vi "10054_Control.vi"(5 "DO":bool caption="DO ON/OFF", 7 "error in":errorcluster, 8 "Operation":T1, 9 "Pin":T2=enum."Pilz-2", 10 "Resource In":refnum<visa-resource-name>) -> (0 "error out":errorcluster, 1 "Status":bool[](array[boolean]), 2 "Command Response":string, 3 "Resource out":refnum<visa-resource-name>)   [LabVIEW 2021]
uses:
  Support/10054_states.ctl
  Support/Relay_no.ctl
panel:
  # "UART TX"
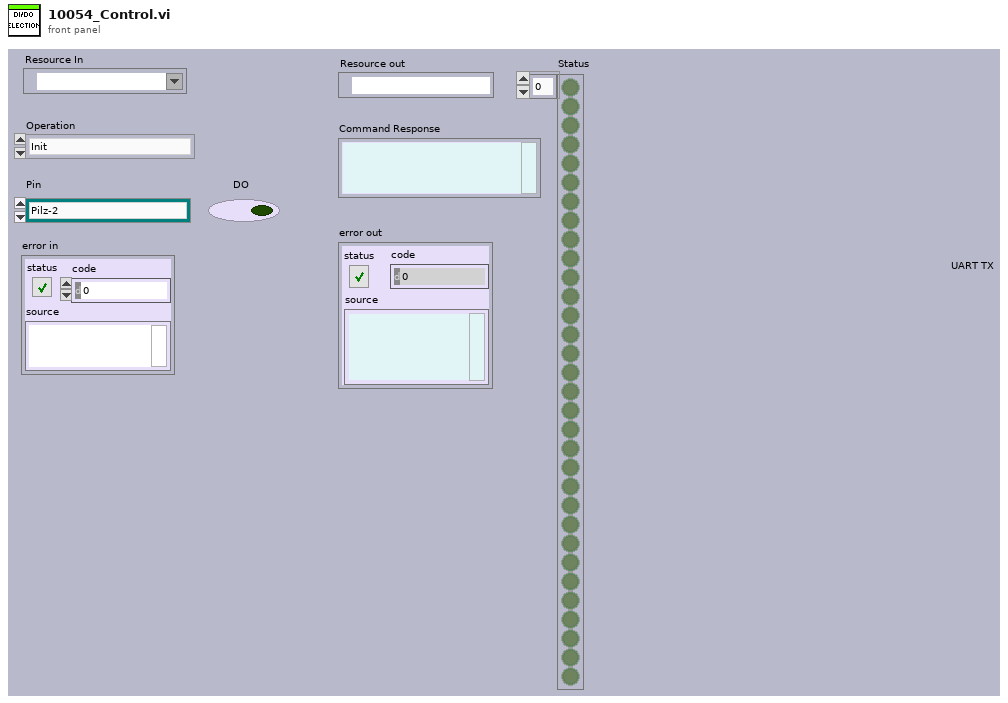
[diagram p1: front panel]
types:
  T1 = typedef "Relay_no.ctl" = enum16{"Init", "write&Read", "PCB Serial Write & Read", "PCB Write SSD & Password", "Read Wifi state", "Reset", "Close"}
  T2 = typedef "10054_states.ctl" = enum16{"Pilz-1", "Pilz-2", "AC CON - 2", "AC CON - 3", "AC CON - 4", "AC CON - 5", "Tower Lamp - Red", "Tower Lamp - Amber", "Tower Lamp - Green", "FAN 1 & 2", "FAN 3 & 4", "FAN 5 & 6", "Load - 1 10A", "Load - 2 10A", "Load - 3 5A", "Load - 4 5A", "Load - 5 2A", "TP49 - 12V", "TP20 - 5V", "TP148 - 3.3", "TP193 - GND", "J11.1 POS", "J11.2 NEG", "Noti LED POS", "Noti LED NEG", "Noti LED  5V", "D+M J14.1 - 3.3", "D+M J14.2 - GND", "NFC - 1", "NFC - 2"}
  T3 = cluster{"baud rate":u32, "data bits":u16, "parity":enum16{"None", "Odd", "Even", "Mark", "Space"}, "stop bits":u16, "flow control":u16}
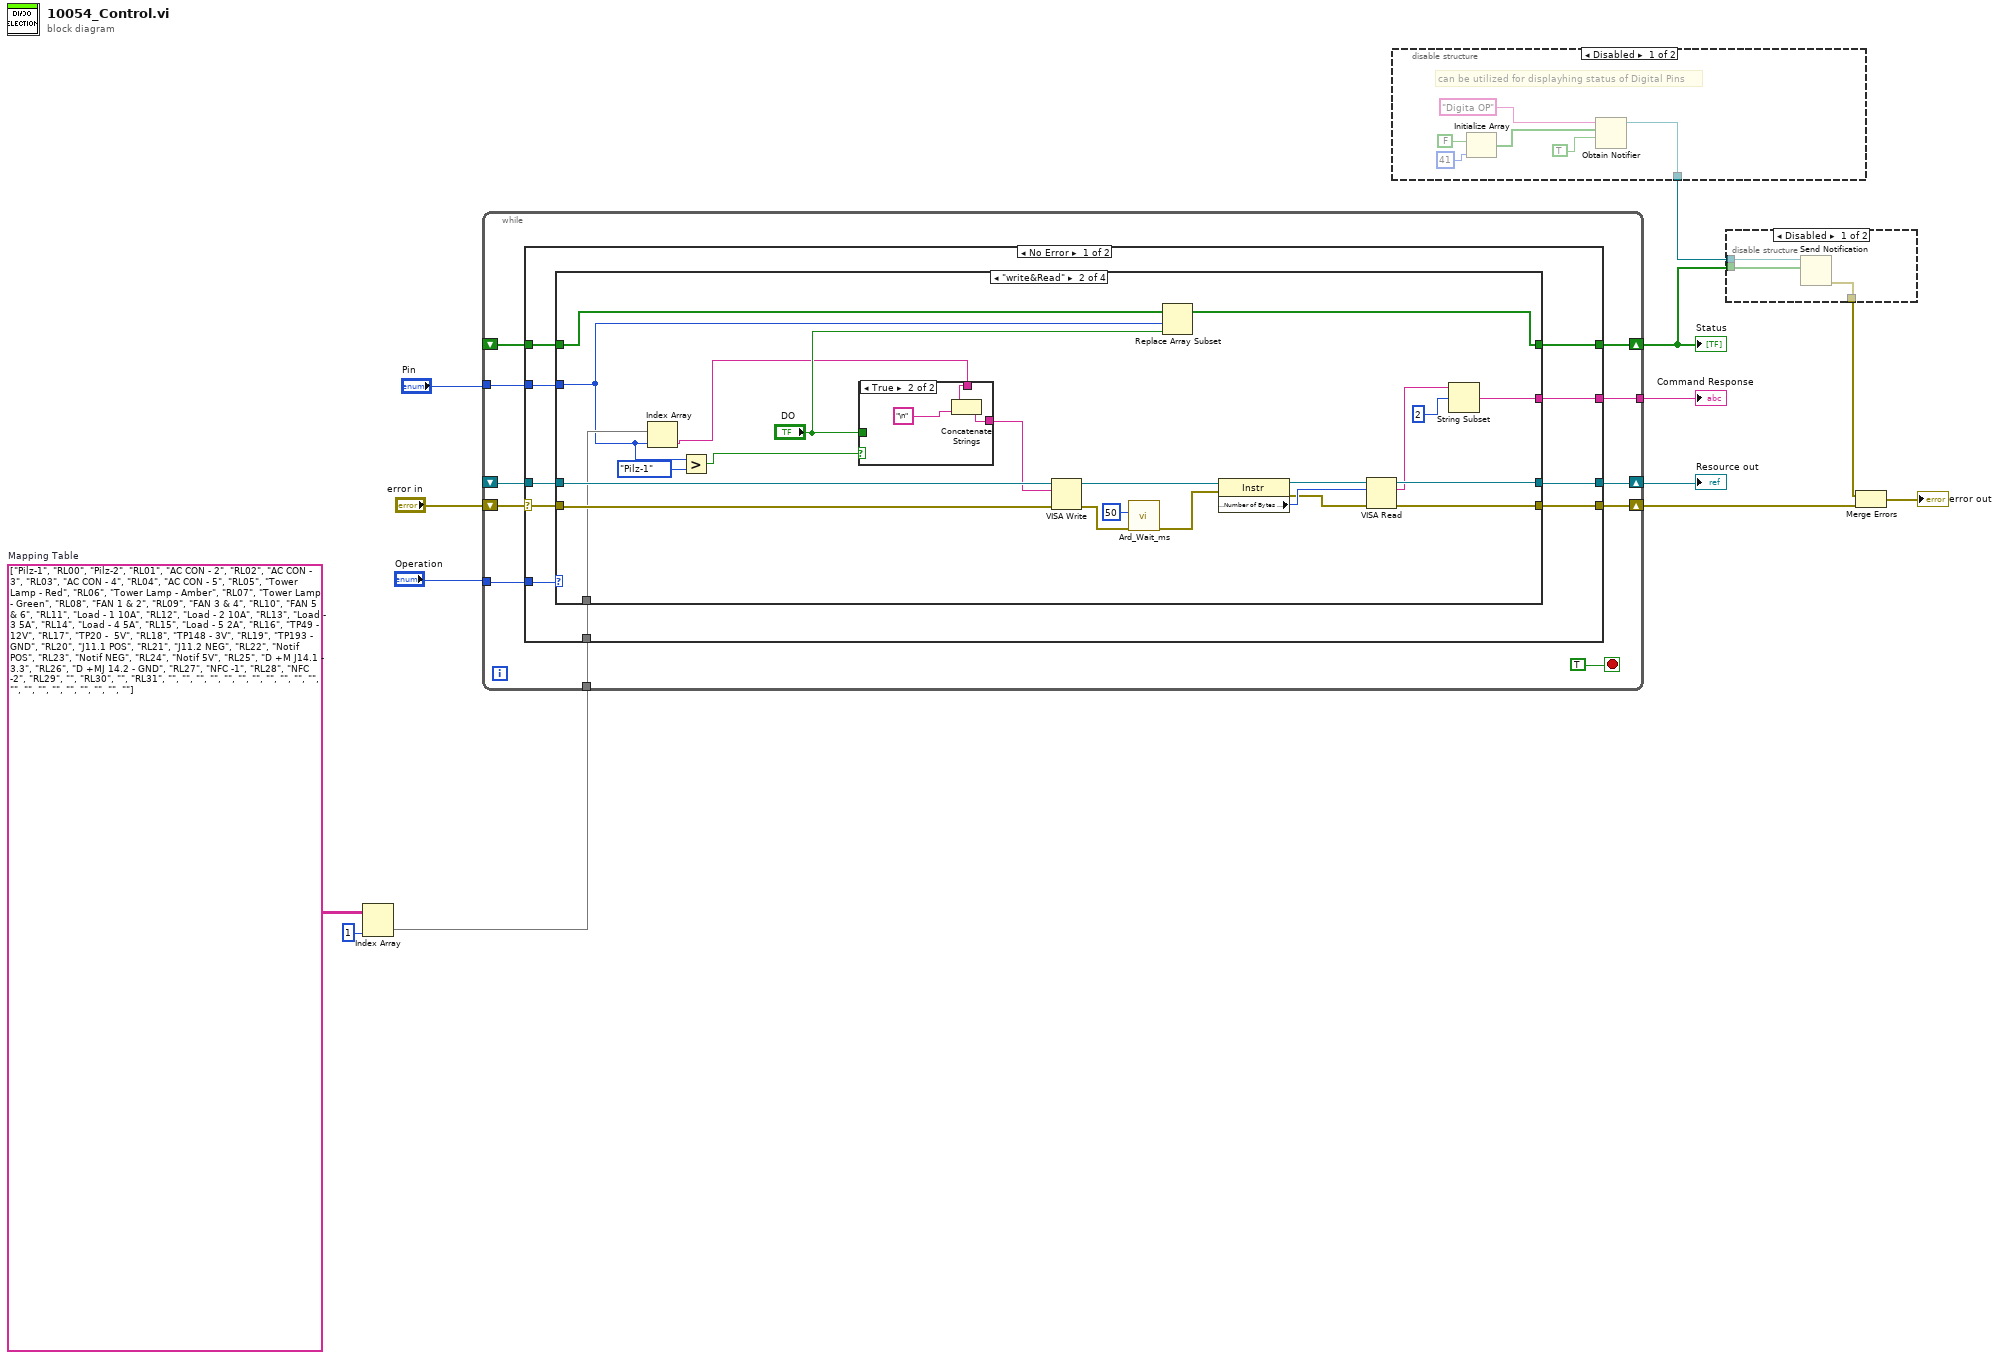
[diagram p0: block diagram]
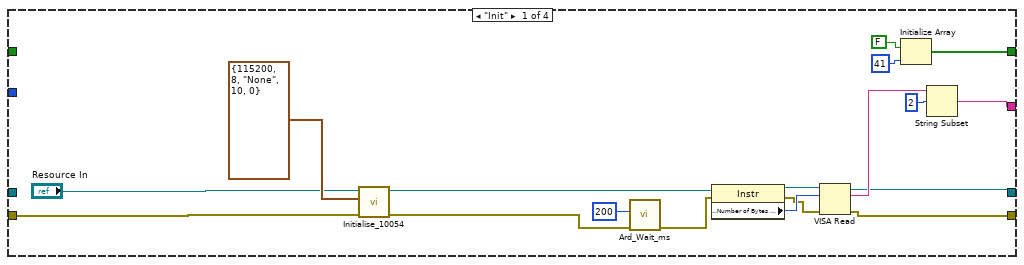
[diagram p4: hidden frame]
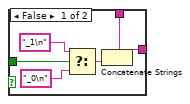
[diagram p5: hidden frame]
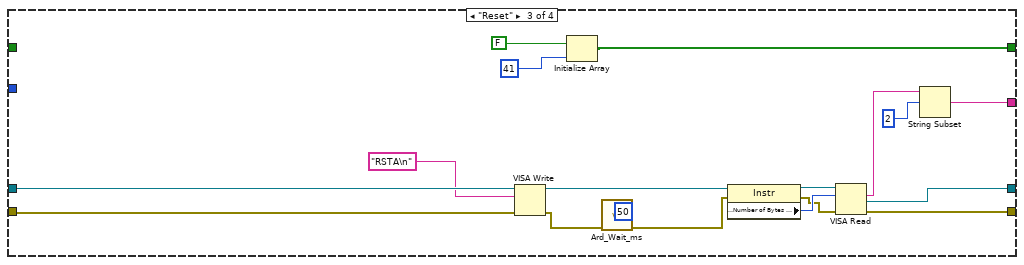
[diagram p6: hidden frame]
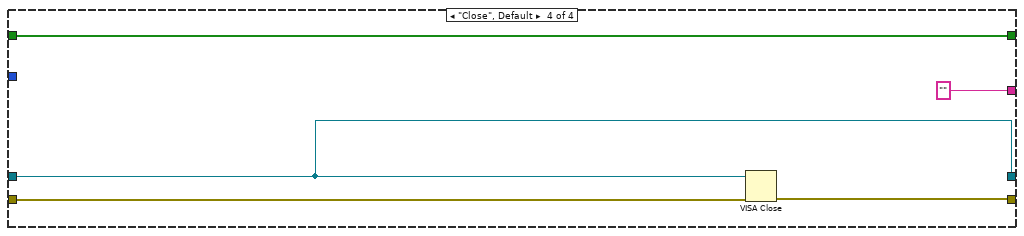
[diagram p7: hidden frame]
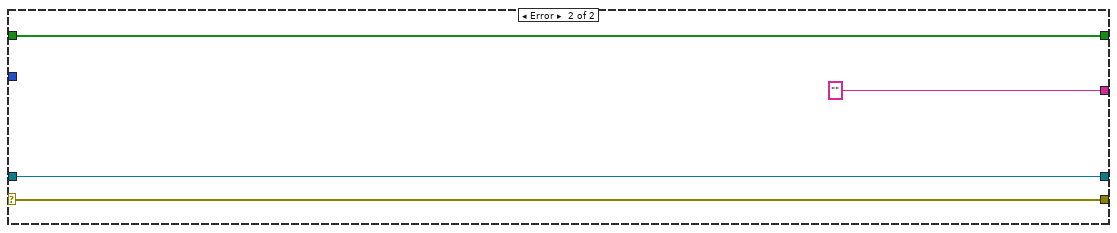
[diagram p8: hidden frame]
diagram:
  w5 = string[][] [["Pilz-1", "RL00"], ["Pilz-2", "RL01"], ["AC CON - 2", "RL02"], ["AC CON - 3", "RL03"], ["AC CON - 4", "RL04"], ["AC CON - 5", "RL05"], ["Tower Lamp - Red", "RL06"], ["Tower Lamp - Amber", "RL07"], ["Tower Lamp - Green", "RL08"], ["FAN 1 & 2", "RL09"], ["FAN 3 & 4", "RL10"], ["FAN 5 & 6", "RL11"], ["Load - 1 10A", "RL12"], ["Load - 2 10A", "RL13"], ["Load - 3 5A", "RL14"], ["Load - 4 5A", "RL15"], ["Load - 5 2A", "RL16"], ["TP49 - 12V", "RL17"], ["TP20 -  5V", "RL18"], ["TP148 - 3V", "RL19"], ["TP193 - GND", "RL20"], ["J11.1 POS", "RL21"], ["J11.2 NEG", "RL22"], ["Notif POS", "RL23"], ["Notif NEG", "RL24"], ["Notif 5V", "RL25"], ["D +M J14.1 - 3.3", "RL26"], ["D +MJ 14.2 - GND", "RL27"], ["NFC -1", "RL28"], ["NFC -2", "RL29"], ["", "RL30"], ["", "RL31"], ["", ""], ["", ""], ["", ""], ["", ""], ["", ""], ["", ""], ["", ""], ["", ""], ["", ""], ["", ""]]  # Mapping Table
  n1 = Index Array(array=w5, index (col)=1 ("disabled index (col)")) -> (element=w3:string[])  [unwired: 1 in]
  n2 = while {
    tunnel: "Operation" -> [w23]
    shift-right: [w22] -> w11
    shift-left: _ -> [w20]
    shift-right: [w21] -> w9
    shift-left: "error in" -> [w19]
    tunnel: [w18] -> w12
    shift-right: [w16] -> w10
    shift-left: _ -> [w17]
    tunnel: "Pin" -> [w15]
    tunnel: w3 -> [w14]
    stop <- TRUE stop-if-true
    n3 = case shown="No Error" w19 {
      selector: w19 -> [w30 w108]
      tunnel: w23 -> [w34 _]
      tunnel: [w33 w110] -> w22
      tunnel: [w32 w108] -> w21
      tunnel: w20 -> [w31 w110]
      tunnel: [w29 "" ("read buffer")] -> w18
      tunnel: w17 -> [w28 w107]
      tunnel: [w27 w107] -> w16
      tunnel: w15 -> [w26 _]
      tunnel: w14 -> [w25 _]
      frame No Error {
        n4 = case shown="\"write&Read\"" w34 {
          tunnel: [w43 w70 w96 w105] -> w33
          tunnel: w30 -> [w50 w59 w89 w103]
          tunnel: [w41 w71 w97 w102] -> w32
          tunnel: w31 -> [_ w75 w101 w105]
          tunnel: [w42 w64 w90 "" ("read buffer")] -> w29
          tunnel: w28 -> [_ w62 _ w104]
          tunnel: [w38 w60 w85 w104] -> w27
          tunnel: w26 -> [_ w55 _ _]
          tunnel: w25 -> [_ w58 _ _]
          frame "Init" {
            n5 = call "Initialise_10054 .vi"("error in"=w50, "Serial Settings"=T3 {"baud rate"=115200, "data bits"=8, "parity"=enum."None", "stop bits"=10, "flow control"=0}, "RS232 name in"="Resource In") -> ("error out"=w36:errorcluster, "RS232 name out"=w35:refnum<visa-resource-name>)  [unwired: 7 in]
            n6 = call "Ard_Wait_ms.vi"("error in"=w36, "millisec"=u32 200) -> ("error in 2"=w46:errorcluster)  [unwired: 9 in]
            n7 = property class="Instr"(reference=w35, error in=w46) -> (reference out=w47:refnum<visa-resource-name>, error out=w48:errorcluster, "Serial Settings:Number of Bytes at Serial Port"=w49:u32)
            n8 = VISA Read(VISA resource name=w47, byte count=w49, error in (no error)=w48) -> (VISA resource name out=w43:refnum<visa-resource-name>, read buffer=w45:string, error out=w41:errorcluster)  [unwired: 1 out]
            n9 = Initialize Array(FALSE, 41 ("dimension size")) -> (w38:bool[])
            n10 = String Subset(string=w45, offset (0)=2) -> (substring=w42:string)  [unwired: 1 in]
          }
          frame "write&Read" {
            n11 = Index Array(array=w58, index=w55) -> (element=w57:string)
            n12 = Greater?(x=w55, y=10054_states."Pilz-1") -> (0:w53:bool)
            n13 = case shown="True" w53 {
              tunnel: [w81 w83] -> w63
              tunnel: "DO" -> [w80 _]
              tunnel: w57 -> [w79 w84]
              frame False {
                n14 = Select(t="_1\n", s=w80, f="_0\n") -> (s? t:f=w76:string)
                n15 = Concatenate Strings(w79, w76) -> (w81:string)
              }
              frame True {
                n16 = Concatenate Strings(w84, "\n") -> (w83:string)
              }
            }
            n17 = VISA Write(VISA resource name=w75, write buffer=w63, error in (no error)=w59) -> (VISA resource name out=w69:refnum<visa-resource-name>, error out=w68:errorcluster)  [unwired: 1 out]
            n18 = call "Ard_Wait_ms.vi"("error in"=w68, "millisec"=u32 50) -> ("error in 2"=w67:errorcluster)  [unwired: 9 in]
            n19 = Replace Array Subset(array=w62, new element="DO", index=w55) -> (w60:bool[])
            n20 = property class="Instr"(reference=w69, error in=w67) -> (reference out=w72:refnum<visa-resource-name>, error out=w73:errorcluster, "Serial Settings:Number of Bytes at Serial Port"=w74:u32)
            n21 = VISA Read(VISA resource name=w72, byte count=w74, error in (no error)=w73) -> (VISA resource name out=w70:refnum<visa-resource-name>, read buffer=w66:string, error out=w71:errorcluster)  [unwired: 1 out]
            n22 = String Subset(string=w66, offset (0)=2) -> (substring=w64:string)  [unwired: 1 in]
          }
          frame "Reset" {
            (unwired) u32 50 ("millisec")
            n23 = VISA Write(VISA resource name=w101, write buffer="RSTA\n", error in (no error)=w89) -> (VISA resource name out=w95:refnum<visa-resource-name>, error out=w94:errorcluster)  [unwired: 1 out]
            n24 = Initialize Array(FALSE, 41 ("dimension size")) -> (w85:bool[])
            n25 = call "Ard_Wait_ms.vi"("error in"=w94) -> ("error in 2"=w93:errorcluster)  [unwired: 10 in]
            n26 = property class="Instr"(reference=w95, error in=w93) -> (reference out=w98:refnum<visa-resource-name>, error out=w99:errorcluster, "Serial Settings:Number of Bytes at Serial Port"=w100:u32)
            n27 = VISA Read(VISA resource name=w98, byte count=w100, error in (no error)=w99) -> (VISA resource name out=w96:refnum<visa-resource-name>, read buffer=w92:string, error out=w97:errorcluster)  [unwired: 1 out]
            n28 = String Subset(string=w92, offset (0)=2) -> (substring=w90:string)  [unwired: 1 in]
          }
          frame "Close", Default {
            n29 = VISA Close(VISA resource name=w105, error in (no error)=w103) -> (error out=w102:errorcluster)
          }
        }
      }
      frame Error {
      }
    }
  }
  "Command Response" <- w12
  "Resource out" <- w11
  "Status" <- w10
  n30 = disable-structure shown="Disabled" {
    disable-tunnel: [w111 _] -> w7
    frame Disabled {
      # "can be utilized for displayhing status of Digital Pins"
      n31 = Initialize Array(FALSE, 41 ("dimension size")) -> (w112:bool[])
      n32 = Obtain Notifier(name (unnamed)="Digita OP", notification data type=w112, create if not found? (T)=TRUE) -> (notifier out=w111:refnum<notifier>)  [unwired: 1 in, 2 out]
    }
    frame Enabled {
    }
  }
  n33 = disable-structure shown="Disabled" {
    disable-tunnel: w10 -> [w119 _]
    disable-tunnel: w7 -> [w118 _]
    disable-tunnel: [w117 _] -> w6
    frame Disabled {
      n34 = Send Notification(notification=w119, notifier=w118) -> (error out=w117:errorcluster)  [unwired: 1 in, 1 out]
    }
    frame Enabled {
    }
  }
  n35 = Merge Errors(w6, w9) -> (→"error out":errorcluster)
